vi "query Reference Level.vi"(8 "error in (no error)":errorcluster, 11 "FSV-40N in":refnum<class "FSV-40N.lvclass">) -> (0 "error out":errorcluster, 2 "Ref Level":dbl, 3 "FSV-40N out":refnum<class "FSV-40N.lvclass">)   [LabVIEW 2023, in "Spectrum Analyzer.lvlib" / "FSV-40N.lvclass"]
uses:
  FSV-40N.lvclass
  FSV-40N.lvclass/FSV-40N.ctl
  Spectrum Analyzer.lvlib
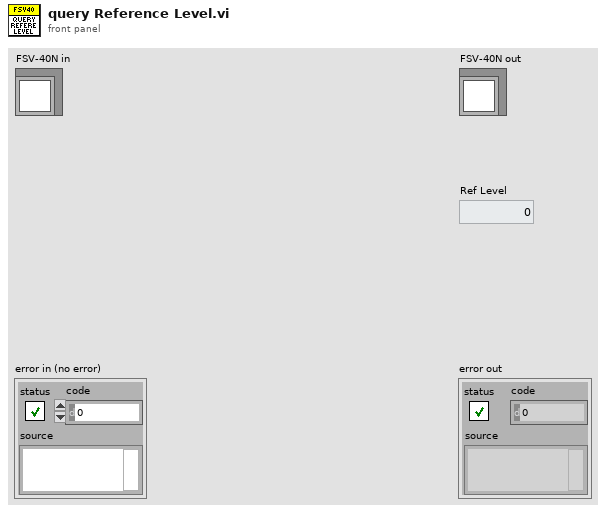
[diagram p1: front panel]
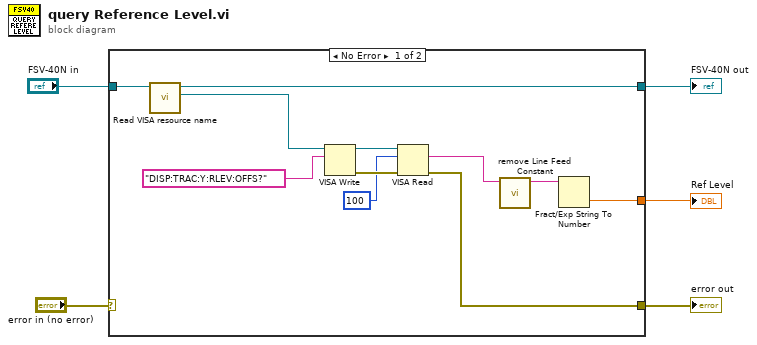
[diagram p0: block diagram]
diagram:
  n1 = case shown="No Error" "error in (no error)" {
    selector: "error in (no error)" -> [_ w17]
    tunnel: "FSV-40N in" -> [w16 w18]
    tunnel: [w14 w18] -> w4
    tunnel: [w9 w17] -> w2
    tunnel: [w6 _] -> w1
    frame No Error {
      n2 = call "Read VISA resource name.vi"("FSV-40N in"=w16) -> ("VISA resource name"=w15:refnum<visa-resource-name>, "FSV-40N out"=w14:refnum<class "FSV-40N.lvclass">)  [unwired: 8 in, 1 out]
      n3 = VISA Write(VISA resource name=w15, write buffer="DISP:TRAC:Y:RLEV:OFFS?") -> (VISA resource name out=w12:refnum<visa-resource-name>, error out=w11:errorcluster)  [unwired: 1 in, 1 out]
      n4 = VISA Read(VISA resource name=w12, byte count=u32 100, error in (no error)=w11) -> (read buffer=w8:string, error out=w9:errorcluster)  [unwired: 2 out]
      n5 = call "remove Line Feed Constant.vi"("Input String"=w8) -> ("Line Feed Removed String"=w7:string)  [unwired: 10 in]
      n6 = Fract/Exp String To Number(string=w7) -> (number=w6:dbl)  [unwired: 3 in, 1 out]
    }
    frame Error {
    }
  }
  "error out" <- w2
  "FSV-40N out" <- w4
  "Ref Level" <- w1
